vi "MQTT Subscriptions - Handle Suback.vi"(0 "MQTT ref in":T1, 5 "Packet ID":u16, 7 "Reason Codes":u8[](array[numeric]), 9 "Reason String":string) -> (4 "MQTT ref out":T1)   [LabVIEW 2019, in "KoRE-MQTT.lvlib"]
doc: "Copyright (c) 2025 KoRElibs.com\nSPDX-License-Identifier: EUPL-1.2\n\nThis VI is licensed under the European Union Public License (EUPL) Version 1.2. You may use this VI unmodified in proprietary works. If you distribute a modified version of this file, the modified file must be released under the EUPL-1.2. Full license: https://joinup.ec.europa.eu/asset/eupl/eupl/1.2/"
uses:
  KoRE-MQTT.lvlib
  Public/TypeDefs/MQTT Client Session.ctl
  TypeDefs/MQTT Client Session - Data Value Reference.ctl
  Public/TypeDefs/MQTT Client Session - Data.ctl
  Public/TypeDefs/MQTT Property - Will.ctl
  Public/TypeDefs/MQTT Property - CONNECT.ctl
  TypeDefs/MQTT Subscription - Info.ctl
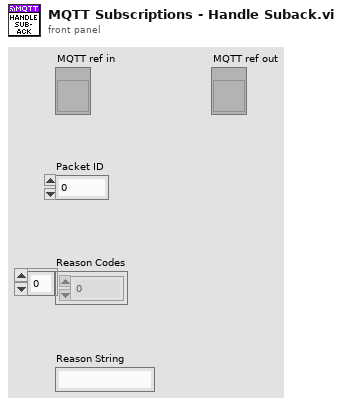
[diagram p1: front panel]
types:
  T1 = typedef "KoRE-MQTT.lvlib/MQTT Client Session.ctl" = refnum<vi>
  T2 = typedef "KoRE-MQTT.lvlib/MQTT Client Session - Data Value Reference.ctl" = refnum<data-value>
  T3 = typedef "KoRE-MQTT.lvlib/MQTT Client Session - Data.ctl" = cluster{"TCP ref":refnum<k5>, "Next Packet Id":u16, "Version":u8, "Host":string, "Port":u16, "Ping Delta":u32, "Username":string, "Password":string, "Will QoS":u8, "Will Retain":bool, "Will Topic":string, "Will Payload":string, "TCP Timeout":i32, "Semaphore":T4, "In-Flight Messages":variant, "Close":bool, "Last Send":u32, "Keep Alive":u16, "Last Ping RTT":u32, "Last Ping":u32, "Will Properties":T5[], "Session Expiry Interval":u32, "Maximum QoS":u8, "Retain Available":bool, "Server Maximum Packet Size":u32, "Client Identifier":string, "Server Topic Alias Maximum":u16, "Wildcard Subscription Available":bool, "Subscription Identifier Available":bool, "Shared Subscription Available":bool, "Connect Properties":T6[], "Client Maximum Packet Size":u32, "Client Topic Alias Maximum":u16, "Server Receive Maximum":u16, "Client Receive Maximum":u16, "TLS cfg":refnum<k36>, "Subscriptions":T7[]}
  T4 = typedef "Semaphore RefNum" = refnum<k1>
  T5 = typedef "KoRE-MQTT.lvlib/MQTT Property - Will.ctl" = cluster{"Property":u8, "Value":string}
  T6 = typedef "KoRE-MQTT.lvlib/MQTT Property - CONNECT.ctl" = cluster{"Property":u8, "Value":string}
  T7 = typedef "KoRE-MQTT.lvlib/MQTT Subscription - Info.ctl" = cluster{"Packet Id":u16, "Index":u16, "Identifier":u32, "QoS":u8, "Topic Filter":string, "Reason Code":u8, "Reason String":string, "Granted":bool}
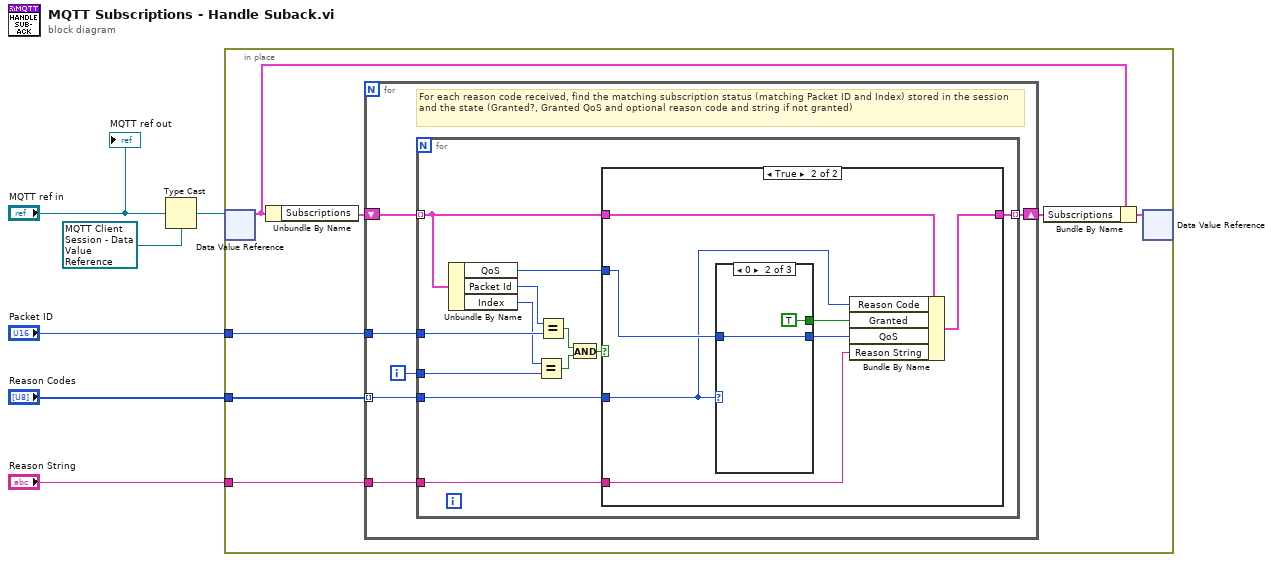
[diagram p0: block diagram]
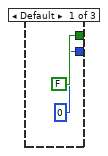
[diagram p3: hidden frame]
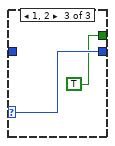
[diagram p4: hidden frame]
diagram:
  n1 = Type Cast(type=T2 refnum ("data value reference"), x="MQTT ref in") -> (*(type *) &x=w3:T2)
  n2 = in-place {
    in-place-border: "Packet ID" -> [w13]
    in-place-border: "Reason Codes" -> [w12]
    in-place-border: "Reason String" -> [w7]
    n3 = in-place-dvr #1(w3) -> (w8:T3)  [unwired: 1 out]
    n4 = Unbundle By Name(w8) -> ("Subscriptions"=w11:T7[])
    n5 = for {
      tunnel: w13 -> [w19]
      tunnel: w12 -> [w15] mode=indexing
      shift-right: [w16] -> w10
      shift-left: w11 -> [w17]
      tunnel: w7 -> [w14]
      i -> [w18]
      # "For each reason code received, find the matching subscription status (matching Packet ID and Index) stored in the session and the state (Granted?, Granted QoS and optional reason code and string if not granted)"
      n6 = for {
        tunnel: w17 -> [w24] mode=indexing
        tunnel: w19 -> [w30]
        tunnel: w18 -> [w28]
        tunnel: [w23] -> w16 mode=indexing
        tunnel: w15 -> [w22]
        tunnel: w14 -> [w21]
        n7 = Unbundle By Name(w24) -> ("QoS"=w20:u8, "Packet Id"=w31:u16, "Index"=w29:u16)
        n8 = Equal?(x=w29, y=w28) -> (x = y?=w27:bool)
        n9 = Equal?(x=w31, y=w30) -> (x = y?=w26:bool)
        n10 = And(x=w26, y=w27) -> (x .and. y?=w25:bool)
        n11 = case shown="True" w25 {
          tunnel: w24 -> [w32 w39]
          tunnel: [w32 w38] -> w23
          tunnel: w22 -> [_ w33]
          tunnel: w21 -> [_ w35]
          tunnel: w20 -> [_ w34]
          frame False {
          }
          frame True {
            n12 = case shown="0" w33 {
              selector: w33 -> [_ _ w45]
              tunnel: [u8 0 w43 w45] -> w37
              tunnel: [FALSE TRUE TRUE] -> w36
              tunnel: w34 -> [_ w43 _]
              frame Default {
              }
              frame 0 {
              }
              frame 1, 2 {
              }
            }
            n13 = Bundle By Name(cluster=w39, "Reason Code"=w33, "Granted"=w36, "QoS"=w37, "Reason String"=w35) -> (w38:T7)
          }
        }
      }
    }
    n14 = Bundle By Name(cluster=w8, "Subscriptions"=w10) -> (w9:T3)
    n15 = in-place-dvr #1(w9) -> ()  [unwired: 2 out]
  }
  "MQTT ref out" <- "MQTT ref in"
